vi "test Parameter Add-Find-Remove.vi"(8 "error in":errorcluster, 11 "TestCase in":refnum<class "Scripting.lvclass">) -> (0 "error out":errorcluster, 3 "TestCase out":refnum<class "Scripting.lvclass">)   [LabVIEW 2023, in "Scripting.lvclass"]
uses:
  Scripting.lvclass
  Scripting.lvclass/Scripting.ctl
  <vilib>/addons/_JKI Toolkits/VI Tester/TestCase.llb/TestCase.lvclass
  Scripting/Ballard/Ballard ARINC 429 Scripting.lvlib
  Shared/Direction.ctl
  <vilib>/NI VeriStand/Custom Device API/Custom Device Item Ref.ctl
  <vilib>/NI VeriStand/Custom Device API/Custom Device API.lvlib
  Shared/SDI.ctl
  <vilib>/NI/NI VeriStand Encoding and Decoding/Encoding.ctl
  <vilib>/NI/NI VeriStand Encoding and Decoding/Encoding and Decoding.lvlib
  Shared/Parameter Definition.ctl
  Shared/Transfer Speed.ctl
  C:/Program Files/National Instruments/LabVIEW 2025/vi.lib/addons/_JKI Toolkits/VI Tester/TestCase.llb/TestCase.lvclass
  C:/Users/Administrator/Git/niveristand-ballard-arinc429-custom-device/Source/Custom Device Support/Tests/Unit/Scripting/Scripting.lvclass
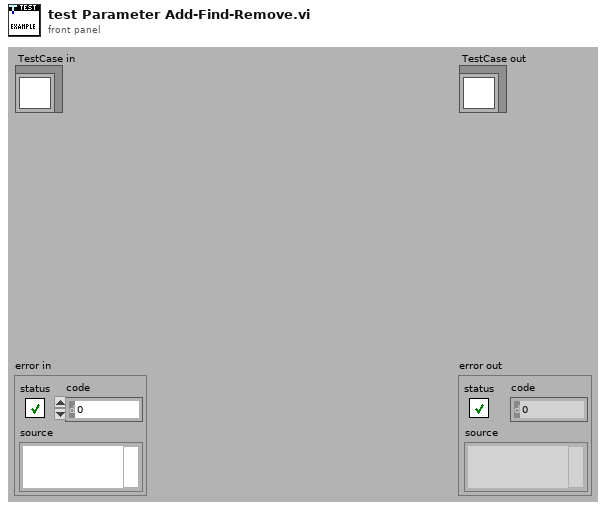
[diagram p1: front panel]
types:
  T1 = typedef "Transfer Speed.ctl" = enum16{"LO (12.5 kb/s)", "HI (100 kb/s)"}
  T2 = cluster{"SDI":bool, "SSM":bool, "Parity":bool, "Timestamp":bool}
  T3 = typedef "Parameter Definition.ctl" = cluster{"start index":i32, "size":i32, "encoding":T4, "signed":bool, "scale multiplier":dbl, "scale offset":dbl}
  T4 = typedef "Encoding and Decoding.lvlib/Encoding.ctl" = enum16{"BNR", "BCD", "Discrete"}
  T5 = typedef "Direction.ctl" = enum16{"Rx", "Tx"}
  T6 = typedef "Custom Device API.lvlib/Custom Device Item Ref.ctl" = u64
  T7 = cluster{"name":string, "unit":string, "default value":dbl}
  T8 = typedef "SDI.ctl" = i32
  T9 = typedef "Custom Device API.lvlib/Custom Device Channel.ctl" = cluster{"Type":T10, "Units":string, "Default Value":dbl, "Faultable":bool, "Scalable":bool}
  T10 = typedef "Custom Device API.lvlib/Custom Device Channel Type.ctl" = enum16{"Input", "Output"}
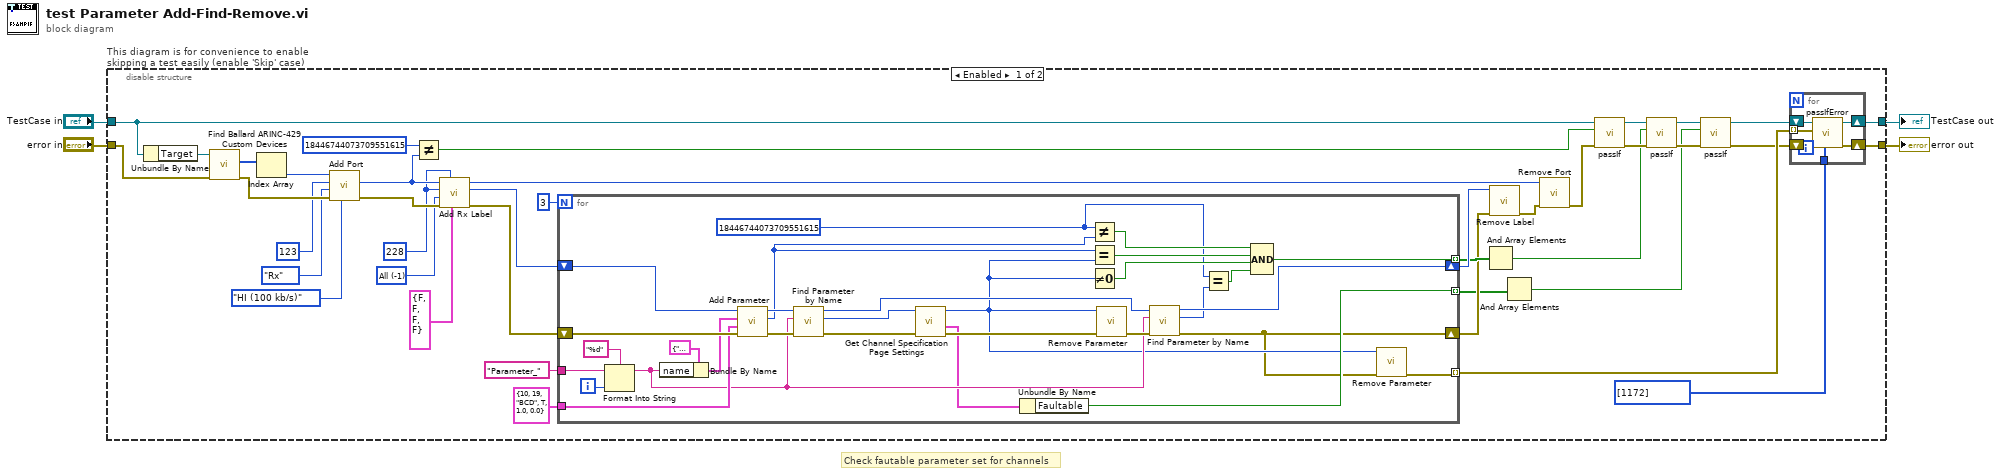
[diagram p0: block diagram]
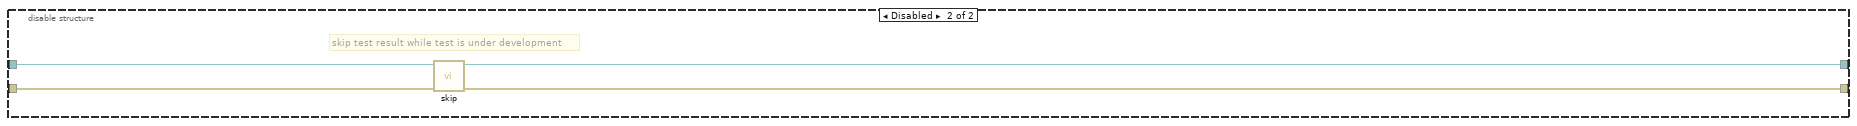
[diagram p2: hidden frame]
diagram:
  # "Check fautable parameter set for channels"
  n1 = disable-structure "This diagram is for convenience to enable skipping a test easily (enable 'Skip' case)" shown="Enabled" {
    disable-tunnel: "TestCase in" -> [w41 w84]
    disable-tunnel: [w17 w82] -> w1
    disable-tunnel: [w18 w83] -> w3
    disable-tunnel: "error in" -> [w43 w81]
    frame Enabled {
      w11 = u32 228 ("label value")
      w37 = T8 -1 items=["All"=-1, "0 (b00)"=0, "1 (b01)"=1, "2 (b10)"=2, "3 (b11)"=3] ("SDI value")
      n2 = Unbundle By Name(w41) -> ("Target"=w44:refnum<k24>)
      n3 = call "Find Ballard ARINC-429 Custom Devices.vi"("error in"=w43, "target in"=w44) -> ("error out"=w35:errorcluster, "Ballard ARINC 429 custom devices"=w42:u64[])  [unwired: 7 in, 1 out]
      n4 = Index Array(array=w42) -> (element=w36:u64)  [unwired: 1 in]
      n5 = call "Add Port.vi"("speed (HI 100 kb/s)"=Transfer_Speed."HI (100 kb/s)" ("speed"), "error in"=w35, "direction"=Direction."Rx", "port number"=u16 123, "Ballard ARINC 429 custom device in"=w36) -> ("error out"=w40:errorcluster, "port"=w12:T6)  [unwired: 4 in, 1 out]
      n6 = Not Equal?(x=T6 18446744073709551615 ("custom device ref out"), y=w12) -> (x != y?=w31:bool)
      n7 = call "Add Rx Label.vi"("create channels"=T2 {"SDI"=FALSE, "SSM"=FALSE, "Parity"=FALSE, "Timestamp"=FALSE}, "label (Display)"=w11, "error in"=w40, "SDI value"=w37, "label (Dec)"=w11, "port in"=w12) -> ("error out"=w25:errorcluster, "label"=w27:T6, "port out"=w39:T6)  [unwired: 3 in]
      n8 = for {
        N: 3 -> [_]
        shift-right: [w64] -> w26
        shift-left: w27 -> [w57]
        shift-right: [w51] -> w21
        shift-left: w25 -> [w76]
        tunnel: T3 {"start index"=10, "size"=19, "encoding"=enum."BCD", "signed"=TRUE, "scale multiplier"=1.0, "scale offset"=0.0} ("parameter definition") -> [w75]
        tunnel: "Parameter_" ("initial string") -> [w72]
        tunnel: [w65] -> w22 mode=indexing
        tunnel: [w61] -> w19 mode=indexing
        tunnel: [w59] -> w5 mode=indexing
        i -> [w73]
        w63 = T6 18446744073709551615 ("custom device ref out")
        n9 = Format Into String(format string="%d", initial string=w72, w73) -> (resulting string=w69:string)  [unwired: 1 in, 1 out]
        n10 = Bundle By Name(cluster=T7 {"name"="", "unit"="super units", "default value"=3.0} ("parameter"), "name"=w69) -> (w70:T7)
        n11 = call "Add Parameter.vi"("error in"=w76, "parameter encoding"=w75, "parameter definition"=w70, "label in"=w57) -> ("error out"=w77:errorcluster, "parameter"=w58:T6, "label out"=w80:T6)  [unwired: 5 in]
        n12 = call "Find Parameter by Name.vi"("error in"=w77, "parameter name"=w69, "label in"=w80) -> ("error out"=w56:errorcluster, "parameter ref"=w54:T6, "label out"=w78:T6)  [unwired: 5 in, 1 out]
        n13 = call "Get Channel Specification Page Settings.vi"("error in"=w56, "parameter ref"=w54) -> ("error out"=w55:errorcluster, "Channel"=w52:T9, "parameter ref out"=w53:T6)  [unwired: 6 in, 1 out]
        n14 = Unbundle By Name(w52) -> ("Faultable"=w59:bool)
        n15 = Not Equal?(x=w63, y=w58) -> (x != y?=w67:bool)
        n16 = Equal?(x=w58, y=w53) -> (x = y?=w68:bool)
        n17 = Not Equal To 0?(x=w53) -> (x != 0?=w66:bool)
        n18 = call "Remove Parameter.vi"("error in"=w55, "parameter"=w53) -> ("error out"=w79:errorcluster)  [unwired: 9 in]
        n19 = call "Find Parameter by Name.vi"("error in"=w79, "parameter name"=w69, "label in"=w78) -> ("error out"=w51:errorcluster, "parameter ref"=w60:T6, "label out"=w64:T6)  [unwired: 5 in, 1 out]
        n20 = Equal?(x=w63, y=w60) -> (x = y?=w62:bool)
        n21 = Compound Arithmetic op=AND(w67, w68, w66, w62) -> (w65:bool)
        n22 = call "Remove Parameter.vi"("error in"=w51, "parameter"=w53) -> ("error out"=w61:errorcluster)  [unwired: 9 in]
      }
      n23 = And Array Elements(Boolean array=w22) -> (logical AND=w20:bool)
      n24 = call "Remove Label.vi"("error in"=w21, "label"=w26) -> ("error out"=w30:errorcluster)  [unwired: 9 in]
      n25 = And Array Elements(Boolean array=w5) -> (logical AND=w8:bool)
      n26 = call "Remove Port.vi"("error in"=w30, "port"=w39) -> ("error out"=w15:errorcluster)  [unwired: 9 in]
      n27 = call-dynamic "passIf.vi"("error in (no error)"=w15, "pass"=w31, "TestCase in"=w41) -> ("error out"=w29:errorcluster, "TestCase out"=w38:refnum<class "Scripting.lvclass">)  [unwired: 7 in]
      n28 = call-dynamic "passIf.vi"("error in (no error)"=w29, "pass"=w20, "TestCase in"=w38) -> ("error out"=w10:errorcluster, "TestCase out"=w9:refnum<class "Scripting.lvclass">)  [unwired: 7 in]
      n29 = call-dynamic "passIf.vi"("error in (no error)"=w10, "pass"=w8, "TestCase in"=w9) -> ("error out"=w6:errorcluster, "TestCase out"=w7:refnum<class "Scripting.lvclass">)  [unwired: 7 in]
      n30 = for {
        tunnel: w19 -> [w50] mode=indexing
        shift-right: [w47] -> w17
        shift-left: w7 -> [w48]
        shift-right: [w46] -> w18
        shift-left: w6 -> [w49]
        tunnel: i32[] [1172] ("passing error codes (default = any error code)") -> [w45]
        n31 = call-dynamic "passIfError.vi"("passing error codes (default = any error code)"=w45, "error in (no error)"=w49, "error"=w50, "TestCase in"=w48) -> ("error out"=w46:errorcluster, "TestCase out"=w47:refnum<class "Scripting.lvclass">)  [unwired: 6 in]
      }
    }
    frame Disabled {
      # "skip test result while test is under development"
      n32 = call <vilib>:"skip.vi"("error in (no error)"=w81, "TestCase in"=w84) -> ("error out"=w83:errorcluster, "TestCase out"=w82:refnum<class "Scripting.lvclass">)  [unwired: 8 in]
    }
  }
  "error out" <- w3
  "TestCase out" <- w1
